vi "ReadSymbolCatalog.vi"(8 "error in (no error)":errorcluster, 11 "AdsNET in":refnum<class "AdsNET.lvclass">) -> (0 "error out":errorcluster, 3 "AdsNET out":refnum<class "AdsNET.lvclass">, 4 "Elapsed Time (ms)":u32)   [LabVIEW 2016, in "TCatAdsNet.lvlib" / "AdsNET.lvclass"]
doc: "Reads symbol names and properties."
uses:
  AdsNET.lvclass
  AdsNET.lvclass/AdsNET.ctl
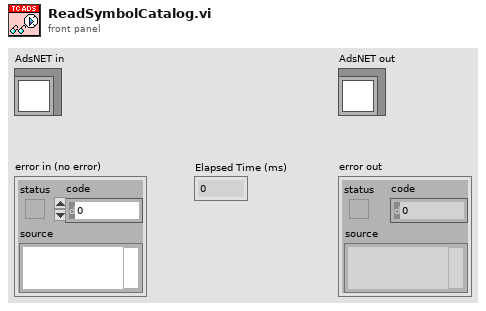
[diagram p1: front panel]
types:
  T1 = cluster{"Name":string, "IndexGroup":i64, "IndexOffset":i64, "Size":i32, "Type":string, "Datatype":i32, "Comment":string}
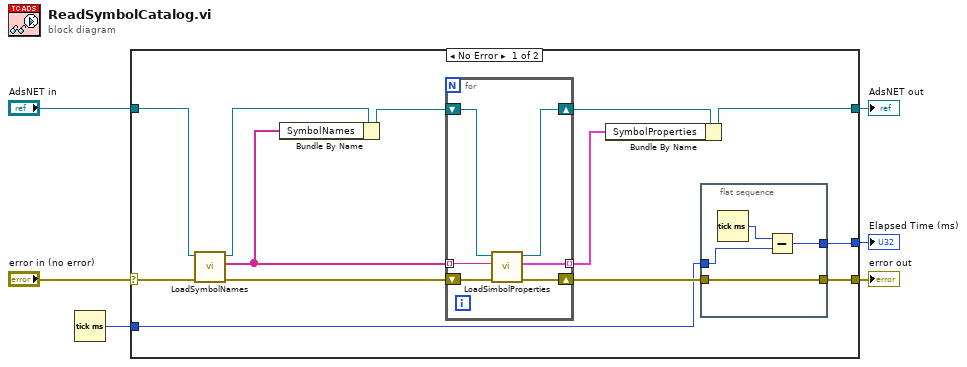
[diagram p0: block diagram]
diagram:
  n1 = Tick Count (ms)() -> (millisecond timer value=w2:u32)
  n2 = case shown="No Error" "error in (no error)" {
    selector: "error in (no error)" -> [w17 w31]
    tunnel: [w9 w31] -> w5
    tunnel: [w12 w30] -> w3
    tunnel: "AdsNET in" -> [w19 w30]
    tunnel: w2 -> [w8 _]
    tunnel: [w7 _] -> w1
    frame No Error {
      n3 = call "LoadSymbolNames.vi"("error in (no error)"=w17, "TCatAdsNet in"=w19) -> ("error out"=w14:errorcluster, "SymbolNameList"=w13:string[], "TCatAdsNet out"=w18:refnum<class "AdsNET.lvclass">)  [unwired: 7 in]
      n4 = Bundle By Name(cluster=w18, "SymbolNames"=w13) -> (w16:refnum<class "AdsNET.lvclass">)
      n5 = for {
        shift-right: [w28] -> w15
        shift-left: w16 -> [w29]
        shift-right: [w26] -> w10
        shift-left: w14 -> [w27]
        tunnel: w13 -> [w25] mode=indexing
        tunnel: [w24] -> w11 mode=indexing
        n6 = call "LoadSimbolProperties.vi"("error in (no error)"=w27, "name"=w25, "TCatAdsNet in"=w29) -> ("error out"=w26:errorcluster, "SymbolProperties"=w24:T1, "TCatAdsNet out"=w28:refnum<class "AdsNET.lvclass">)  [unwired: 5 in, 1 out]
      }
      n7 = Bundle By Name(cluster=w15, "SymbolProperties"=w11) -> (w12:refnum<class "AdsNET.lvclass">)
      n8 = flat-sequence {
        tunnel: w10 -> [w23]
        tunnel: [w23] -> w9
        tunnel: w8 -> [w21]
        tunnel: [w20] -> w7
        frame #0 {
          n9 = Tick Count (ms)() -> (millisecond timer value=w22:u32)
          n10 = Subtract(x=w22, y=w21) -> (x-y=w20:u32)
        }
      }
    }
    frame Error {
    }
  }
  "error out" <- w5
  "AdsNET out" <- w3
  "Elapsed Time (ms)" <- w1
